vi "Test Launcher DebugTerminal.vi"   [LabVIEW 2013]
uses:
  Stream Direction -- enum.ctl
  <vilib>/LabVIEW Open Source Project/MQTT Control Packets/Control Packets/CONNECT/Create CONNECT Packet.vi
  Process_OutgoingOnly.vi
  Process_All_single.vi
  DebuggingTerminal.lvclass
  <vilib>/LabVIEW Open Source Project/MQTT Control Packets/Control Packets/DISCONNECT/DISCONNECT.lvclass
  <vilib>/LabVIEW Open Source Project/MQTT Control Packets/Control Packets/PUBLISH/PUBLISH.lvclass
  <vilib>/LabVIEW Open Source Project/MQTT Control Packets/Control Packets/PINGREQ/PINGREQ.lvclass
  <vilib>/LabVIEW Open Source Project/MQTT Control Packets/Control Packets/CONNACK/CONNACK.lvclass
  <vilib>/LabVIEW Open Source Project/MQTT Control Packets/Control Packets/PINGRESP/PINGRESP.lvclass
  <vilib>/LabVIEW Open Source Project/MQTT Control Packets/Control Packets/PUBACK/PUBACK.lvclass
  <vilib>/LabVIEW Open Source Project/MQTT Control Packets/Control Packets/PUBREC/PUBREC.lvclass
  <vilib>/LabVIEW Open Source Project/MQTT Control Packets/Control Packets/PUBREL/PUBREL.lvclass
  <vilib>/LabVIEW Open Source Project/MQTT Control Packets/Control Packets/PUBCOMP/PUBCOMP.lvclass
  <vilib>/LabVIEW Open Source Project/MQTT Control Packets/Control Packets/CONNECT/CONNECT.lvclass
  MQTT Base.lvlib
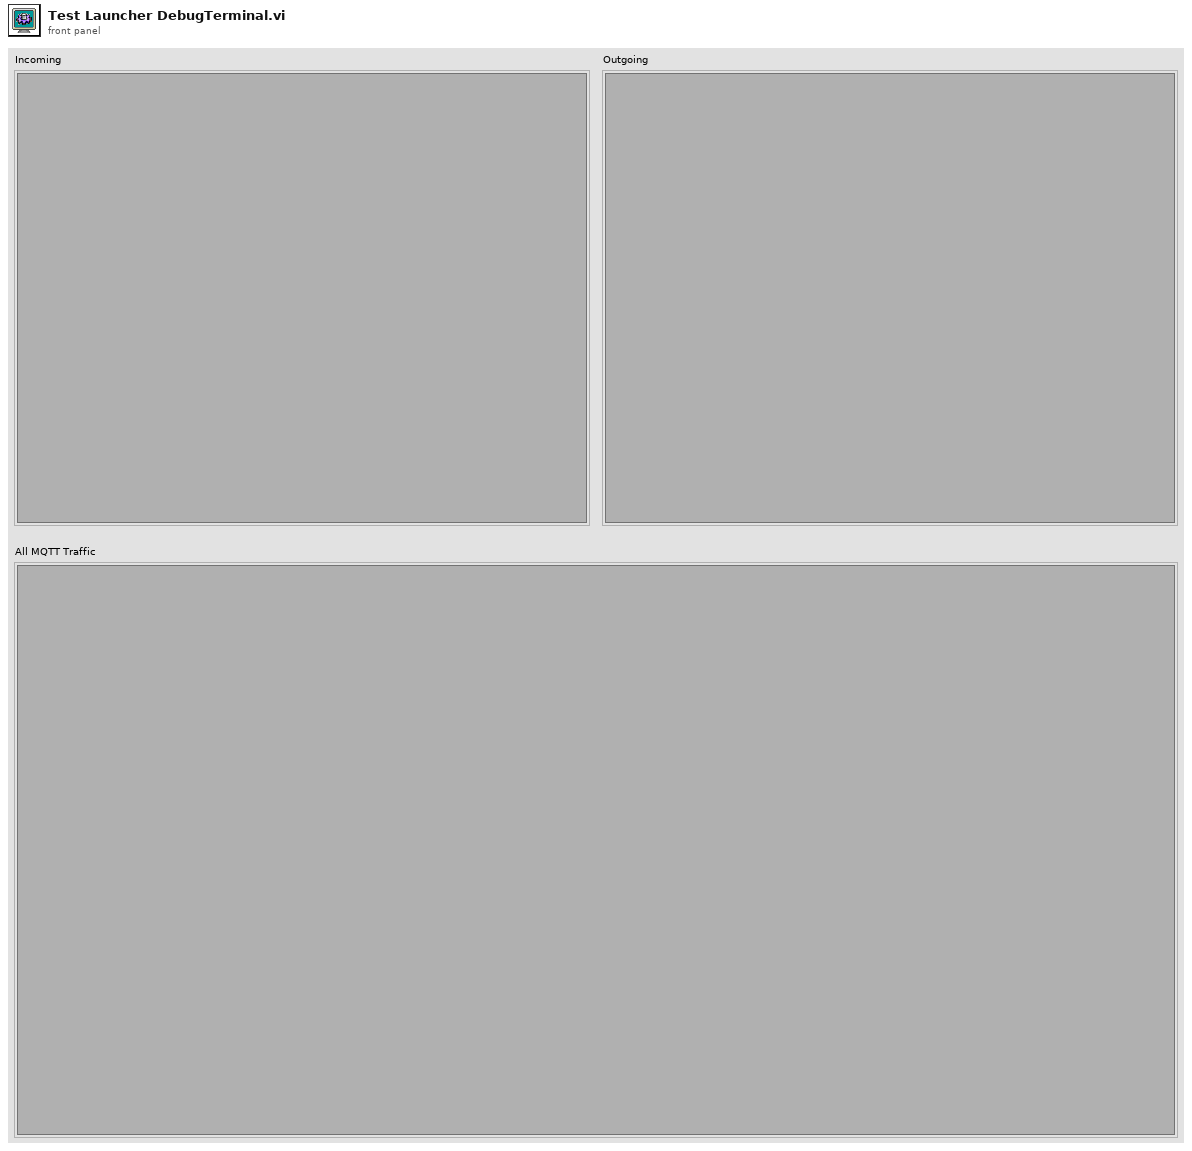
[diagram p1: front panel]
types:
  T1 = typedef "MQTT Base.lvlib/DebuggingTerminal.lvclass/Stream Direction -- enum.ctl" = enum16{"Incoming", "Outgoing"}
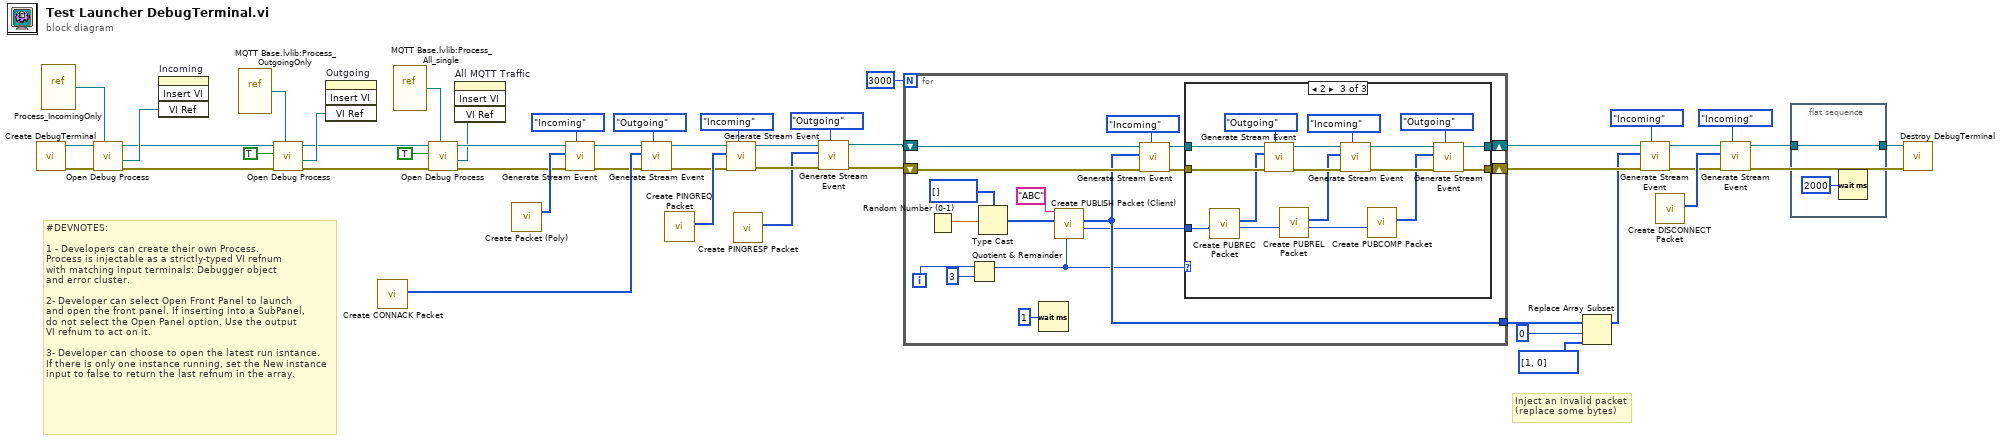
[diagram p0: block diagram]
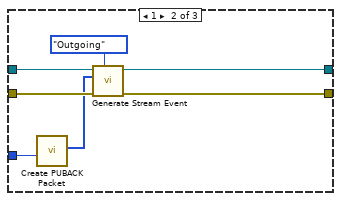
[diagram p3: hidden frame]
diagram:
  # "#DEVNOTES: \n\n1 - Developers can create their own Process. \nProcess is injectable as a strictly-typed VI refnum\nwith matching input terminals: Debugger object\nand error cluster.\n\n2- Developer can select Open Front Panel to launch\nand open the front panel. If inserting into a SubPanel,\ndo not select the Open Panel option. Use the output\nVI refnum to act on it.\n\n3- Developer can choose to open the latest run isntance.\nIf there is only one instance running, set the New instance\ninput to false to return the last refnum in the array."
  # "Inject an invalid packet\n(replace some bytes)"
  n1 = call "Create DebugTerminal.vi"() -> ("error out"=w46:errorcluster, "DebuggingTerminal out"=w47:refnum<class "DebuggingTerminal.lvclass">)  [unwired: 10 in]
  n2 = vi-ref "Process_IncomingOnly.vi"() -> (w13:refnum<vi>)
  n3 = call "Open Debug Process.vi"("Process"=w13, "error in (no error)"=w46, "DebuggingTerminal in"=w47) -> ("error out"=w11:errorcluster, "VI Refnum"=w14:refnum<vi>, "DebuggingTerminal out"=w12:refnum<class "DebuggingTerminal.lvclass">)  [unwired: 6 in]
  n4 = invoke on="Incoming" class="SubPanel" method="Insert VI"("VI Ref"=w14) -> ()  [unwired: 3 in, 4 out]
  n5 = vi-ref "MQTT Base.lvlib:Process_OutgoingOnly.vi"() -> (w8:refnum<vi>)
  n6 = call "Open Debug Process.vi"("Process"=w8, "error in (no error)"=w11, "New instance?"=TRUE, "DebuggingTerminal in"=w12) -> ("error out"=w4:errorcluster, "VI Refnum"=w10:refnum<vi>, "DebuggingTerminal out"=w5:refnum<class "DebuggingTerminal.lvclass">)  [unwired: 5 in]
  n7 = invoke on="Outgoing" class="SubPnl" method="Insert VI"("VI Ref"=w10) -> ()  [unwired: 3 in, 4 out]
  n8 = call <vilib>:"Create CONNACK Packet.vi"() -> ("Bytes Stream"=w25:u8[])  [unwired: 9 in, 2 out]
  n9 = vi-ref "MQTT Base.lvlib:Process_All_single.vi"() -> (w7:refnum<vi>)
  n10 = call "Open Debug Process.vi"("Process"=w7, "error in (no error)"=w4, "New instance?"=TRUE, "DebuggingTerminal in"=w5) -> ("error out"=w3:errorcluster, "VI Refnum"=w1:refnum<vi>, "DebuggingTerminal out"=w2:refnum<class "DebuggingTerminal.lvclass">)  [unwired: 5 in]
  n11 = invoke on="All MQTT Traffic" class="SubPnl" method="Insert VI"("VI Ref"=w1) -> ()  [unwired: 3 in, 4 out]
  n12 = call-poly <vilib>:"Create Packet (Poly).vi"() -> ("Bytes Stream"=w43:u8[])  [unwired: 9 in, 2 out]
  n13 = call "Generate Stream Event.vi"("Direction"=Stream_Direction_--_enum."Incoming", "error in (no error)"=w3, "Bytes"=w43, "DebuggingTerminal in"=w2) -> ("error out"=w22:errorcluster, "DebuggingTerminal out"=w24:refnum<class "DebuggingTerminal.lvclass">)  [unwired: 6 in]
  n14 = call "Generate Stream Event.vi"("Direction"=Stream_Direction_--_enum."Outgoing", "error in (no error)"=w22, "Bytes"=w25, "DebuggingTerminal in"=w24) -> ("error out"=w21:errorcluster, "DebuggingTerminal out"=w23:refnum<class "DebuggingTerminal.lvclass">)  [unwired: 6 in]
  n15 = call <vilib>:"Create PINGREQ Packet.vi"() -> ("Bytes Stream"=w38:u8[])  [unwired: 9 in, 2 out]
  n16 = call "Generate Stream Event.vi"("Direction"=Stream_Direction_--_enum."Incoming", "error in (no error)"=w21, "Bytes"=w38, "DebuggingTerminal in"=w23) -> ("error out"=w17:errorcluster, "DebuggingTerminal out"=w19:refnum<class "DebuggingTerminal.lvclass">)  [unwired: 6 in]
  n17 = call <vilib>:"Create PINGRESP Packet.vi"() -> ("Bytes Stream"=w16:u8[])  [unwired: 9 in, 2 out]
  n18 = call "Generate Stream Event.vi"("Direction"=Stream_Direction_--_enum."Outgoing", "error in (no error)"=w17, "Bytes"=w16, "DebuggingTerminal in"=w19) -> ("error out"=w15:errorcluster, "DebuggingTerminal out"=w18:refnum<class "DebuggingTerminal.lvclass">)  [unwired: 6 in]
  n19 = for {
    N: 3000 -> [_]
    shift-right: [w52] -> w35
    shift-left: w18 -> [w64]
    shift-right: [w50] -> w33
    shift-left: w15 -> [w63]
    tunnel: [w54] -> w30
    i -> [w56]
    n20 = Random Number (0-1)() -> (number: 0 to 1=w60:dbl)
    n21 = Quotient & Remainder(x=w56, y=3) -> (x-y*floor(x/y)=w49:i32)  [unwired: 1 out]
    n22 = Type Cast(type=u8[] [] ("Bytes"), x=w60) -> (*(type *) &x=w58:u8[])
    n23 = Wait (ms)(milliseconds to wait=u32 1) -> ()  [unwired: 1 out]
    n24 = call <vilib>:"Create PUBLISH Packet (Client).vi"("QoS"=w49, "Payload"=w58, "Topic Name"="ABC") -> ("Packet ID"=w48:u16, "Bytes Stream"=w54:u8[])  [unwired: 5 in, 2 out]
    n25 = call "Generate Stream Event.vi"("Direction"=Stream_Direction_--_enum."Incoming", "error in (no error)"=w63, "Bytes"=w54, "DebuggingTerminal in"=w64) -> ("error out"=w51:errorcluster, "DebuggingTerminal out"=w53:refnum<class "DebuggingTerminal.lvclass">)  [unwired: 6 in]
    n26 = case shown="2" w49 {
      tunnel: w53 -> [w66 w73 w88]
      tunnel: [w66 w72 w77] -> w52
      tunnel: w51 -> [w65 w71 w87]
      tunnel: [w65 w70 w78] -> w50
      tunnel: w48 -> [_ w68 w75]
      frame 0, Default {
      }
      frame 1 {
        n27 = call <vilib>:"Create PUBACK Packet.vi"("Packet ID"=w68) -> ("Bytes Stream"=w67:u8[])  [unwired: 8 in, 2 out]
        n28 = call "Generate Stream Event.vi"("Direction"=Stream_Direction_--_enum."Outgoing", "error in (no error)"=w71, "Bytes"=w67, "DebuggingTerminal in"=w73) -> ("error out"=w70:errorcluster, "DebuggingTerminal out"=w72:refnum<class "DebuggingTerminal.lvclass">)  [unwired: 6 in]
      }
      frame 2 {
        n29 = call <vilib>:"Create PUBREC Packet.vi"("Packet ID"=w75) -> ("Bytes Stream"=w85:u8[])  [unwired: 8 in, 2 out]
        n30 = call "Generate Stream Event.vi"("Direction"=Stream_Direction_--_enum."Outgoing", "error in (no error)"=w87, "Bytes"=w85, "DebuggingTerminal in"=w88) -> ("error out"=w82:errorcluster, "DebuggingTerminal out"=w83:refnum<class "DebuggingTerminal.lvclass">)  [unwired: 6 in]
        n31 = call <vilib>:"Create PUBREL Packet.vi"("Packet ID"=w75) -> ("Bytes Stream"=w76:u8[])  [unwired: 8 in, 2 out]
        n32 = call "Generate Stream Event.vi"("Direction"=Stream_Direction_--_enum."Incoming", "error in (no error)"=w82, "Bytes"=w76, "DebuggingTerminal in"=w83) -> ("error out"=w79:errorcluster, "DebuggingTerminal out"=w80:refnum<class "DebuggingTerminal.lvclass">)  [unwired: 6 in]
        n33 = call <vilib>:"Create PUBCOMP Packet.vi"("Packet ID"=w75) -> ("Bytes Stream"=w74:u8[])  [unwired: 8 in, 2 out]
        n34 = call "Generate Stream Event.vi"("Direction"=Stream_Direction_--_enum."Outgoing", "error in (no error)"=w79, "Bytes"=w74, "DebuggingTerminal in"=w80) -> ("error out"=w78:errorcluster, "DebuggingTerminal out"=w77:refnum<class "DebuggingTerminal.lvclass">)  [unwired: 6 in]
      }
    }
  }
  n35 = Replace Array Subset(array=w30, new element=u8[] [1, 0] ("Bytes"), index=0) -> (w29:u8[])
  n36 = call "Generate Stream Event.vi"("Direction"=Stream_Direction_--_enum."Incoming", "error in (no error)"=w33, "Bytes"=w29, "DebuggingTerminal in"=w35) -> ("error out"=w32:errorcluster, "DebuggingTerminal out"=w34:refnum<class "DebuggingTerminal.lvclass">)  [unwired: 6 in]
  n37 = call <vilib>:"Create DISCONNECT Packet.vi"() -> ("Bytes Stream"=w40:u8[])  [unwired: 9 in, 2 out]
  n38 = call "Generate Stream Event.vi"("Direction"=Stream_Direction_--_enum."Incoming", "error in (no error)"=w32, "Bytes"=w40, "DebuggingTerminal in"=w34) -> ("error out"=w41:errorcluster, "DebuggingTerminal out"=w36:refnum<class "DebuggingTerminal.lvclass">)  [unwired: 6 in]
  n39 = flat-sequence {
    tunnel: [w90] -> w37
    tunnel: w36 -> [w90]
    frame #0 {
      n40 = Wait (ms)(milliseconds to wait=u32 2000) -> ()  [unwired: 1 out]
    }
  }
  n41 = call "Destroy DebugTerminal.vi"("error in (no error)"=w41, "DebuggingTerminal in"=w37) -> ()  [unwired: 8 in, 2 out]
